vi "IDN.vi"(6 "timeout (ms) [100]":i32=100, 8 "error in (no error)":errorcluster, 11 "Instrument in":refnum<class "Instrument.lvclass">) -> (0 "error out":errorcluster, 2 "IDN":T1, 3 "Instrument in":refnum<class "Instrument.lvclass">)   [LabVIEW 2019, in "Instrument.lvlib" / "Instrument.lvclass"]
doc: "Send \"HELP\" command to get API supported by remote Instrument."
uses:
  Instrument.lvclass
  Typedefs/Instrument.IDN--cluster.ctl
  Typedefs/Instrument.Commands--Enum.ctl
  414e67f7-d63b-4b54-9d53-3147801d2a92.vi
  414e67f7-d63b-4b54-9d53-3147801d2a92.vi/38f1c053-643f-45e3-8e5c-6d0ca5cea375.vi
  414e67f7-d63b-4b54-9d53-3147801d2a92.vi/dcaff4ab-748b-4c89-97b4-50c5e72d0494.vi
  <vilib>/Utility/Data Type/Get Type Information.vi
  <vilib>/JDP Science/JSONtext/JSON text to Variant.vi
  <vilib>/JDP Science/JSONtext/LVClass Serializer/JSONtext LVClass Serializer.lvclass
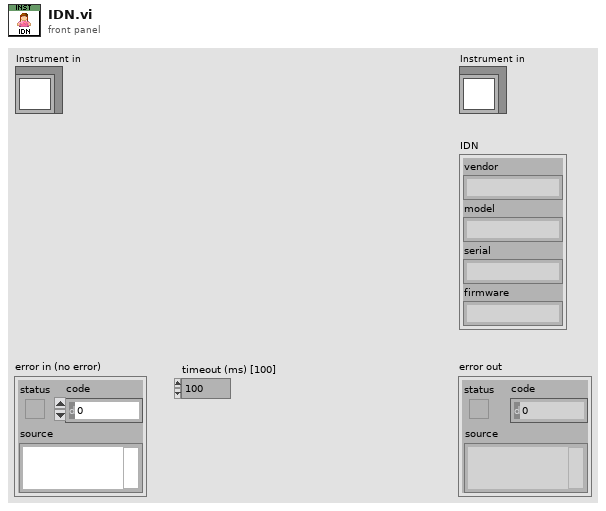
[diagram p1: front panel]
types:
  T1 = typedef "Instrument.lvlib/Instrument.lvclass/Instrument.IDN--cluster.ctl" = cluster{"vendor":string, "model":string, "serial":string, "firmware":string}
  T2 = typedef "Instrument.lvlib/Instrument.lvclass/Instrument.Commands--Enum.ctl" = enum16{"ACK", "HELP", "IDN", "getAll", "getAllData"}
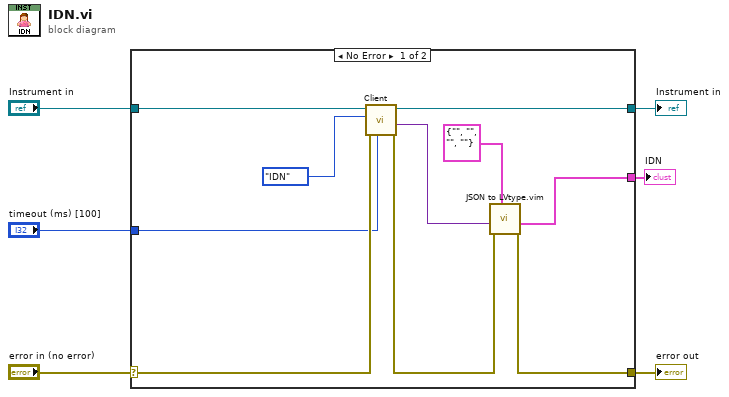
[diagram p0: block diagram]
diagram:
  n1 = case shown="No Error" "error in (no error)" {
    selector: "error in (no error)" -> [w14 w18]
    tunnel: [w11 w18] -> w5
    tunnel: [w16 w17] -> w3
    tunnel: "Instrument in" -> [w15 w17]
    tunnel: [w9 _] -> w2
    tunnel: "timeout (ms) [100]" -> [w7 _]
    frame No Error {
      n2 = call-dynamic "Client.vi"("timeout (ms) [500]"=w7, "error in (no error)"=w14, "Command in"=Instrument.Commands--Enum."IDN" ("Commands"), "Instrument in"=w15) -> ("error out"=w12:errorcluster, "Data out"=w10:variant, "Instrument out"=w16:refnum<class "Instrument.lvclass">)  [unwired: 4 in, 1 out]
      n3 = call "JSON to LVtype.vim"("type"=T1 {"vendor"="", "model"="", "serial"="", "firmware"=""} ("IDN"), "error in (no error)"=w12, "JSON Data in"=w10) -> ("error out"=w11:errorcluster, "Data out"=w9:T1)  [unwired: 7 in]
    }
    frame Error {
    }
  }
  "error out" <- w5
  "Instrument in" <- w3
  "IDN" <- w2
